vi "DSS-Tests-golden_elements.vi"(8 "abs tol":dbl, 9 "rel tol":dbl=1e-12, 10 "golden":dbl[](array[numeric]), 11 "actual":dbl[](array[numeric])) -> (2 "rel diff":dbl[](array[numeric]), 3 "element ok":bool[](array[boolean]))   [LabVIEW 2020, in "DSS-Tests.lvlib"]
doc: "Element by element check of an actual against a golden 1D DBL array: an element is ok when equal, both NaN, or within rel tol times the larger magnitude plus abs tol; also returns each element's relative difference (0 where equal or both NaN)."
uses:
  DSS-Tests.lvlib
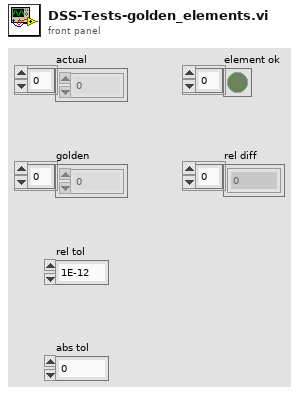
[diagram p1: front panel]
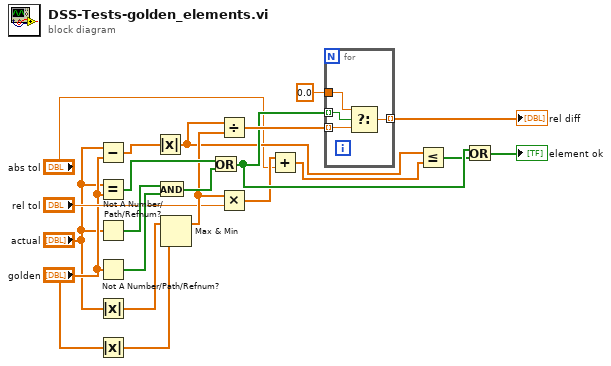
[diagram p0: block diagram]
diagram:
  n1 = Subtract(x="actual", y="golden") -> (x-y=w5:dbl[])
  n2 = Equal?(x="actual", y="golden") -> (x = y?=w13:bool[])
  n3 = Not A Number/Path/Refnum?(number/path/refnum="actual") -> (NaN/Path/Refnum?=w14:bool[])
  n4 = Not A Number/Path/Refnum?(number/path/refnum="golden") -> (NaN/Path/Refnum?=w15:bool[])
  n5 = Absolute Value(x="actual") -> (abs(x)=w7:dbl[])
  n6 = Absolute Value(x="golden") -> (abs(x)=w8:dbl[])
  n7 = Absolute Value(x=w5) -> (abs(x)=w6:dbl[])
  n8 = And(x=w14, y=w15) -> (x .and. y?=w16:bool[])
  n9 = Max & Min(x=w7, y=w8) -> (max(x,y)=w9:dbl[])  [unwired: 1 out]
  n10 = Or(x=w13, y=w16) -> (x .or. y?=w17:bool[])
  n11 = Divide(x=w6, y=w9) -> (x/y=w19:dbl[])
  n12 = Multiply(x=w9, y="rel tol") -> (x*y=w10:dbl[])
  n13 = Add(x=w10, y="abs tol") -> (x+y=w11:dbl[])
  n14 = for {
    tunnel: 0.0 ("zero") -> [w24]
    tunnel: w17 -> [w22] mode=indexing
    tunnel: w19 -> [w23] mode=indexing
    tunnel: [w25] -> w21 mode=indexing
    n15 = Select(t=w24, s=w22, f=w23) -> (s? t:f=w25:dbl)
  }
  "rel diff" <- w21
  n16 = Less Or Equal?(x=w6, y=w11) -> (x <= y?=w12:bool[])
  n17 = Or(x=w17, y=w12) -> (x .or. y?=→"element ok":bool[])
